vi "DriveVelocityHeadingFollower.vi"(0 "RobotMotors":T20={"DriveLeftPrimary"={"DeviceStatus"={"status"=FALSE, "code"=0, "source"=""}, "Type"=enum."PWM", "PWM"={"PWM Channel"=enum."PWM 1", "DeadBand"={"Name"="", "maxPositivePwm"=0, "minPositivePwm"=0, "centerPwm"=0, "maxNegativePwm"=0, "minNegativePwm"=0, "angularRange"=0}}, "CAN"={"Device Number"=0, "SetOutput VI Ref"=variant(enum8{"Percent VBus", "Current", "Speed", "Position", "Voltage"} enum."Percent VBus"), "GetOutput VI Ref"=variant(refnum<k1> refnum), "Enable VI Ref"=variant(dbl 12.0), "Disable VI Ref"=variant(enum8{"Percent VBus", "Speed", "Position", "Slave", "Unchanged / Invalid", "Voltage Compensation", "Current", "Motion Profile"} enum."Percent VBus"), "Data"=variant}, "Invert"=FALSE, "DIO PWM"={"PWM \"Enable\" Channel"=enum."Invalid", "DIOChannel"=enum."Invalid", "PWM Rate"=0.0}}, "DriveLeftSecondary1"={"DeviceStatus"={"status"=FALSE, "code"=0, "source"=""}, "Type"=enum."PWM", "PWM"={"PWM Channel"=enum."PWM 1", "DeadBand"={"Name"="", "maxPositivePwm"=0, "minPositivePwm"=0, "centerPwm"=0, "maxNegativePwm"=0, "minNegativePwm"=0, "angularRange"=0}}, "CAN"={"Device Number"=0, "SetOutput VI Ref"=variant(enum8{"Percent VBus", "Current", "Speed", "Position", "Voltage"} enum."Percent VBus"), "GetOutput VI Ref"=variant(refnum<k1> refnum), "Enable VI Ref"=variant(dbl 12.0), "Disable VI Ref"=variant(enum8{"Percent VBus", "Speed", "Position", "Slave", "Unchanged / Invalid", "Voltage Compensation", "Current", "Motion Profile"} enum."Percent VBus"), "Data"=variant}, "Invert"=FALSE, "DIO PWM"={"PWM \"Enable\" Channel"=enum."Invalid", "DIOChannel"=enum."Invalid", "PWM Rate"=0.0}}, "DriveRightPrimary"={"DeviceStatus"={"status"=FALSE, "code"=0, "source"=""}, "Type"=enum."PWM", "PWM"={"PWM Channel"=enum."PWM 1", "DeadBand"={"Name"="", "maxPositivePwm"=0, "minPositivePwm"=0, "centerPwm"=0, "maxNegativePwm"=0, "minNegativePwm"=0, "angularRange"=0}}, "CAN"={"Device Number"=0, "SetOutput VI Ref"=variant(enum8{"Percent VBus", "Current", "Speed", "Position", "Voltage"} enum."Percent VBus"), "GetOutput VI Ref"=variant(refnum<k1> refnum), "Enable VI Ref"=variant(dbl 12.0), "Disable VI Ref"=variant(enum8{"Percent VBus", "Speed", "Position", "Slave", "Unchanged / Invalid", "Voltage Compensation", "Current", "Motion Profile"} enum."Percent VBus"), "Data"=variant}, "Invert"=FALSE, "DIO PWM"={"PWM \"Enable\" Channel"=enum."Invalid", "DIOChannel"=enum."Invalid", "PWM Rate"=0.0}}, "DriveRightSecondary1"={"DeviceStatus"={"status"=FALSE, "code"=0, "source"=""}, "Type"=enum."PWM", "PWM"={"PWM Channel"=enum."PWM 1", "DeadBand"={"Name"="", "maxPositivePwm"=0, "minPositivePwm"=0, "centerPwm"=0, "maxNegativePwm"=0, "minNegativePwm"=0, "angularRange"=0}}, "CAN"={"Device Number"=0, "SetOutput VI Ref"=variant(enum8{"Percent VBus", "Current", "Speed", "Position", "Voltage"} enum."Percent VBus"), "GetOutput VI Ref"=variant(refnum<k1> refnum), "Enable VI Ref"=variant(dbl 12.0), "Disable VI Ref"=variant(enum8{"Percent VBus", "Speed", "Position", "Slave", "Unchanged / Invalid", "Voltage Compensation", "Current", "Motion Profile"} enum."Percent VBus"), "Data"=variant}, "Invert"=FALSE, "DIO PWM"={"PWM \"Enable\" Channel"=enum."Invalid", "DIOChannel"=enum."Invalid", "PWM Rate"=0.0}}, " RightIntake"={"DeviceStatus"={"status"=FALSE, "code"=0, "source"=""}, "Type"=enum."PWM", "PWM"={"PWM Channel"=enum."PWM 1", "DeadBand"={"Name"="", "maxPositivePwm"=0, "minPositivePwm"=0, "centerPwm"=0, "maxNegativePwm"=0, "minNegativePwm"=0, "angularRange"=0}}, "CAN"={"Device Number"=0, "SetOutput VI Ref"=variant(enum8{"Percent VBus", "Current", "Speed", "Position", "Voltage"} enum."Percent VBus"), "GetOutput VI Ref"=variant(refnum<k1> refnum), "Enable VI Ref"=variant(dbl 12.0), "Disable VI Ref"=variant(enum8{"Percent VBus", "Speed", "Position", "Slave", "Unchanged / Invalid", "Voltage Compensation", "Current", "Motion Profile"} enum."Percent VBus"), "Data"=variant}, "Invert"=FALSE, "DIO PWM"={"PWM \"Enable\" Channel"=enum."Invalid", "DIOChannel"=enum."Invalid", "PWM Rate"=0.0}}, "LeftIntake"={"DeviceStatus"={"status"=FALSE, "code"=0, "source"=""}, "Type"=enum."PWM", "PWM"={"PWM Channel"=enum."PWM 1", "DeadBand"={"Name"="", "maxPositivePwm"=0, "minPositivePwm"=0, "centerPwm"=0, "maxNegativePwm"=0, "minNegativePwm"=0, "angularRange"=0}}, "CAN"={"Device Number"=0, "SetOutput VI Ref"=variant(enum8{"Percent VBus", "Current", "Speed", "Position", "Voltage"} enum."Percent VBus"), "GetOutput VI Ref"=variant(refnum<k1> refnum), "Enable VI Ref"=variant(dbl 12.0), "Disable VI Ref"=variant(enum8{"Percent VBus", "Speed", "Position", "Slave", "Unchanged / Invalid", "Voltage Compensation", "Current", "Motion Profile"} enum."Percent VBus"), "Data"=variant}, "Invert"=FALSE, "DIO PWM"={"PWM \"Enable\" Channel"=enum."Invalid", "DIOChannel"=enum."Invalid", "PWM Rate"=0.0}}, "ArmPivot"={"DeviceStatus"={"status"=FALSE, "code"=0, "source"=""}, "Type"=enum."PWM", "PWM"={"PWM Channel"=enum."PWM 1", "DeadBand"={"Name"="", "maxPositivePwm"=0, "minPositivePwm"=0, "centerPwm"=0, "maxNegativePwm"=0, "minNegativePwm"=0, "angularRange"=0}}, "CAN"={"Device Number"=0, "SetOutput VI Ref"=variant(enum8{"Percent VBus", "Current", "Speed", "Position", "Voltage"} enum."Percent VBus"), "GetOutput VI Ref"=variant(refnum<k1> refnum), "Enable VI Ref"=variant(dbl 12.0), "Disable VI Ref"=variant(enum8{"Percent VBus", "Speed", "Position", "Slave", "Unchanged / Invalid", "Voltage Compensation", "Current", "Motion Profile"} enum."Percent VBus"), "Data"=variant}, "Invert"=FALSE, "DIO PWM"={"PWM \"Enable\" Channel"=enum."Invalid", "DIOChannel"=enum."Invalid", "PWM Rate"=0.0}}, "ArmPivot 2 "={"DeviceStatus"={"status"=FALSE, "code"=0, "source"=""}, "Type"=enum."PWM", "PWM"={"PWM Channel"=enum."PWM 1", "DeadBand"={"Name"="", "maxPositivePwm"=0, "minPositivePwm"=0, "centerPwm"=0, "maxNegativePwm"=0, "minNegativePwm"=0, "angularRange"=0}}, "CAN"={"Device Number"=0, "SetOutput VI Ref"=variant(enum8{"Percent VBus", "Current", "Speed", "Position", "Voltage"} enum."Percent VBus"), "GetOutput VI Ref"=variant(refnum<k1> refnum), "Enable VI Ref"=variant(dbl 12.0), "Disable VI Ref"=variant(enum8{"Percent VBus", "Speed", "Position", "Slave", "Unchanged / Invalid", "Voltage Compensation", "Current", "Motion Profile"} enum."Percent VBus"), "Data"=variant}, "Invert"=FALSE, "DIO PWM"={"PWM \"Enable\" Channel"=enum."Invalid", "DIOChannel"=enum."Invalid", "PWM Rate"=0.0}}, "ArmExtend "={"DeviceStatus"={"status"=FALSE, "code"=0, "source"=""}, "Type"=enum."PWM", "PWM"={"PWM Channel"=enum."PWM 1", "DeadBand"={"Name"="", "maxPositivePwm"=0, "minPositivePwm"=0, "centerPwm"=0, "maxNegativePwm"=0, "minNegativePwm"=0, "angularRange"=0}}, "CAN"={"Device Number"=0, "SetOutput VI Ref"=variant(enum8{"Percent VBus", "Current", "Speed", "Position", "Voltage"} enum."Percent VBus"), "GetOutput VI Ref"=variant(refnum<k1> refnum), "Enable VI Ref"=variant(dbl 12.0), "Disable VI Ref"=variant(enum8{"Percent VBus", "Speed", "Position", "Slave", "Unchanged / Invalid", "Voltage Compensation", "Current", "Motion Profile"} enum."Percent VBus"), "Data"=variant}, "Invert"=FALSE, "DIO PWM"={"PWM \"Enable\" Channel"=enum."Invalid", "DIOChannel"=enum."Invalid", "PWM Rate"=0.0}}, "Climber"={"DeviceStatus"={"status"=FALSE, "code"=0, "source"=""}, "Type"=enum."PWM", "PWM"={"PWM Channel"=enum."PWM 1", "DeadBand"={"Name"="", "maxPositivePwm"=0, "minPositivePwm"=0, "centerPwm"=0, "maxNegativePwm"=0, "minNegativePwm"=0, "angularRange"=0}}, "CAN"={"Device Number"=0, "SetOutput VI Ref"=variant(enum8{"Percent VBus", "Current", "Speed", "Position", "Voltage"} enum."Percent VBus"), "GetOutput VI Ref"=variant(refnum<k1> refnum), "Enable VI Ref"=variant(dbl 12.0), "Disable VI Ref"=variant(enum8{"Percent VBus", "Speed", "Position", "Slave", "Unchanged / Invalid", "Voltage Compensation", "Current", "Motion Profile"} enum."Percent VBus"), "Data"=variant}, "Invert"=FALSE, "DIO PWM"={"PWM \"Enable\" Channel"=enum."Invalid", "DIOChannel"=enum."Invalid", "PWM Rate"=0.0}}, "SelfieStick"={"DeviceStatus"={"status"=FALSE, "code"=0, "source"=""}, "Type"=enum."PWM", "PWM"={"PWM Channel"=enum."PWM 1", "DeadBand"={"Name"="", "maxPositivePwm"=0, "minPositivePwm"=0, "centerPwm"=0, "maxNegativePwm"=0, "minNegativePwm"=0, "angularRange"=0}}, "CAN"={"Device Number"=0, "SetOutput VI Ref"=variant(enum8{"Percent VBus", "Current", "Speed", "Position", "Voltage"} enum."Percent VBus"), "GetOutput VI Ref"=variant(refnum<k1> refnum), "Enable VI Ref"=variant(dbl 12.0), "Disable VI Ref"=variant(enum8{"Percent VBus", "Speed", "Position", "Slave", "Unchanged / Invalid", "Voltage Compensation", "Current", "Motion Profile"} enum."Percent VBus"), "Data"=variant}, "Invert"=FALSE, "DIO PWM"={"PWM \"Enable\" Channel"=enum."Invalid", "DIOChannel"=enum."Invalid", "PWM Rate"=0.0}}}, 1 "RobotConfig":T3={"Motors"={"DriveLeftPrimary"={"CAN Address"=1, "Invert"=FALSE, "InvertSensor"=FALSE, "Unit Conversion Factor"=0.0, "Brake Mode"=enum."Override to Brake", "Reverse Limt Switch Mode"=enum."Normally Closed", "Forward Limt Swith Mode"=enum."Normally Closed", "PWM Channel"=enum."Invalid", "Motor Controller Type"=enum."Talon SRX"}, "DriveLeftSecondary1"={"CAN Address"=2, "Invert"=FALSE, "InvertSensor"=FALSE, "Unit Conversion Factor"=0.0, "Brake Mode"=enum."Override to Brake", "Reverse Limt Switch Mode"=enum."Normally Closed", "Forward Limt Swith Mode"=enum."Normally Closed", "PWM Channel"=enum."Invalid", "Motor Controller Type"=enum."Talon SRX"}, "DriveRightPrimary"={"CAN Address"=3, "Invert"=FALSE, "InvertSensor"=FALSE, "Unit Conversion Factor"=0.0, "Brake Mode"=enum."Override to Brake", "Reverse Limt Switch Mode"=enum."Normally Closed", "Forward Limt Swith Mode"=enum."Normally Closed", "PWM Channel"=enum."Invalid", "Motor Controller Type"=enum."Talon SRX"}, "DriveRightSecondary1"={"CAN Address"=4, "Invert"=FALSE, "InvertSensor"=FALSE, "Unit Conversion Factor"=0.0, "Brake Mode"=enum."Override to Brake", "Reverse Limt Switch Mode"=enum."Normally Closed", "Forward Limt Swith Mode"=enum."Normally Closed", "PWM Channel"=enum."Invalid", "Motor Controller Type"=enum."Talon SRX"}, "RightIntake"={"CAN Address"=8, "Invert"=FALSE, "InvertSensor"=FALSE, "Unit Conversion Factor"=0.0, "Brake Mode"=enum."Override to Brake", "Reverse Limt Switch Mode"=enum."Normally Closed", "Forward Limt Swith Mode"=enum."Normally Closed", "PWM Channel"=enum."Invalid", "Motor Controller Type"=enum."Talon SRX"}, "LeftIntake"={"CAN Address"=7, "Invert"=FALSE, "InvertSensor"=FALSE, "Unit Conversion Factor"=0.0, "Brake Mode"=enum."Override to Brake", "Reverse Limt Switch Mode"=enum."Normally Closed", "Forward Limt Swith Mode"=enum."Normally Closed", "PWM Channel"=enum."Invalid", "Motor Controller Type"=enum."Talon SRX"}, "ArmPivot"={"CAN Address"=5, "Invert"=FALSE, "InvertSensor"=FALSE, "Unit Conversion Factor"=0.0, "Brake Mode"=enum."Override to Brake", "Reverse Limt Switch Mode"=enum."Normally Closed", "Forward Limt Swith Mode"=enum."Normally Closed", "PWM Channel"=enum."Invalid", "Motor Controller Type"=enum."Talon SRX"}, "ArmExtend"={"CAN Address"=6, "Invert"=FALSE, "InvertSensor"=FALSE, "Unit Conversion Factor"=0.0, "Brake Mode"=enum."Override to Brake", "Reverse Limt Switch Mode"=enum."Normally Closed", "Forward Limt Swith Mode"=enum."Normally Closed", "PWM Channel"=enum."Invalid", "Motor Controller Type"=enum."Talon SRX"}, "ArmPivot2"={"CAN Address"=9, "Invert"=FALSE, "InvertSensor"=FALSE, "Unit Conversion Factor"=0.0, "Brake Mode"=enum."Override to Brake", "Reverse Limt Switch Mode"=enum."Normally Closed", "Forward Limt Swith Mode"=enum."Normally Closed", "PWM Channel"=enum."Invalid", "Motor Controller Type"=enum."Talon SRX"}, "Climber"={"CAN Address"=10, "Invert"=FALSE, "InvertSensor"=FALSE, "Unit Conversion Factor"=0.0, "Brake Mode"=enum."Override to Brake", "Reverse Limt Switch Mode"=enum."Disabled", "Forward Limt Swith Mode"=enum."Disabled", "PWM Channel"=enum."Invalid", "Motor Controller Type"=enum."Talon SRX"}, "Selfie Stick"={"CAN Address"=11, "Invert"=FALSE, "InvertSensor"=FALSE, "Unit Conversion Factor"=0.0, "Brake Mode"=enum."Override to Brake", "Reverse Limt Switch Mode"=enum."Disabled", "Forward Limt Swith Mode"=enum."Disabled", "PWM Channel"=enum."Invalid", "Motor Controller Type"=enum."Talon SRX"}}, "Sensors"={"IMU"={"Yaw Axis"=enum."Z", "SPI Bus"=enum."SPI MXP", "AHRS Algorithm"=enum."Complementary", "Calibration Time (s)"=3.0, "Calibrate On Open"=TRUE}, "LimitSwitch1"={"DIOChannel"=enum."DIO 0", "Active Low"=FALSE}, "LimitSwitch2"={"DIOChannel"=enum."DIO 1", "Active Low"=FALSE}, "BeamBreak"={"DIOChannel"=enum."DIO 2", "Active Low"=FALSE}, "JeVois"={"Baud Rate"=9600, "Parity"=0, "Data Bits"=8, "Stop Bits"=10, "Termination Char (0xA = '\\n' = LF)"=10, "Enable Termination Char? (T)"=TRUE, "Flow Control"=0, "Timeout Value (ms)"=5000, "Serial Port"=enum."Onboard RS-232"}}, "PID"={"ArmExtend"={"P"=0.0, "I"=0.0, "D"=0.0, "F"=0.0, "IZone"=0.0}, "ArmRotate"={"P"=0.0, "I"=0.0, "D"=0.0, "F"=0.0, "IZone"=0.0}, "Drive"={"P"=0.0, "I"=0.0, "D"=0.0, "F"=0.0, "IZone"=0.0}, "DriveGyro Kp ((in/sec)/deg)"=0.0, "CameraPole"={"P"=0.0, "I"=0.0, "D"=0.0, "F"=0.0, "IZone"=0.0}}, "Solenoids"={"ArmClaw"={"Forward Channel"=enum."Solenoid 0", "Invert"=FALSE, "Reverse Channel"=enum."Solenoid 0"}, "IntakeExtend"={"Forward Channel"=enum."Solenoid 1", "Invert"=FALSE, "Reverse Channel"=enum."Solenoid 0"}, "IntakeOpen"={"Forward Channel"=enum."Solenoid 2", "Invert"=FALSE, "Reverse Channel"=enum."Solenoid 0"}, " Shifter"={"Forward Channel"=enum."Solenoid 3", "Invert"=FALSE, "Reverse Channel"=enum."Solenoid 0"}}, "RobotDimensions "={"Length"=0.0, "Height"=0.0, "HeightOfBumpers"=0.0, "DistanceFromFrameEdgeToPyramid "=0.0, "HeightOfFrameToIntake"=0.0, "EdgeOfFrameToOrigin"=0.0}, "ArmHomePosition"={"Angle (rad)"=0.0, "Radius (in)"=0.0}, "SelfieStickParams"={"Home Height (in)"=0.0, "CruiseVelocity"=0, "MaxAccel"=0, "Low Height (in)"=0.0, "High Height (in)"=0.0, "Mid Height (in)"=0.0}, "Enable Compressor"=TRUE} {"Sensors"."JeVois"."Flow Control" items=["None", "XON/XOFF", "RTS/CTS", "XON/XOFF & RTS/CTS", "DTR/DSR", "XON/XOFF & DTR/DSR"]; "Sensors"."JeVois"."Termination Char (0xA = '\\n' = LF)" format="%.0x"; "Sensors"."JeVois"."Stop Bits" items=["1.0"=10, "1.5"=15, "2.0"=20]; "Sensors"."JeVois"."Parity" items=["None", "Odd", "Even", "Mark", "Space"]}, 2 "IMU DevRef":T1={"DevStatus"={"status"=FALSE, "code"=0, "source"=""}, "Handle"=0, "SPI Bus"=enum."SPI On-Board, CS0", "Device Found"=FALSE, "Device Ready"=FALSE, "Yaw Axis"=enum."Z", "AHRS Algorithm"=enum."Complementary", "Serial"=0, "Lot ID 2"=0, "Lot ID 1"=0, "Bytes Per Sample"=0, "Calibrate On Open?"=FALSE}, 3 "DriveCompleteNotifier":refnum<notifier>, 4 "DriveGyro Kp ((in/sec)/deg)":dbl) -> ()   [LabVIEW 2017]
uses:
  TypeDefs/RobotComponents/RobotMotors.ctl
  <vilib>/Rock Robotics/WPI/MotorControl/WPI_MotorControlDeviceRef.ctl
  <vilib>/Rock Robotics/WPI/MotorControl/WPI_MotorControlType.ctl
  <vilib>/Rock Robotics/SystemInterfaces/DIO/FPGA_DIOPWMChannel.ctl
  <vilib>/Rock Robotics/WPI/PWM/WPI_PWMDeadband.ctl
  <vilib>/Rock Robotics/SystemInterfaces/DIO/FPGA_DIOChannel.ctl
  TypeDefs/ConfigComponents/Config_Robot.ctl
  ArgosLib/Config/ConfigComponents/TypeDefs/Config_Motor.ctl
  <vilib>/Rock Robotics/WPI/ThirdParty/Phoenix-LabVIEW/Motor Controller/Controls/CTRE_Phoenix_MotorControl_NeutralMode.ctl
  <vilib>/Rock Robotics/WPI/ThirdParty/Phoenix-LabVIEW/Motor Controller/Controls/CTRE_Phoenix_MotorControl_LimitSwitchNormal.ctl
  ArgosLib/Config/ConfigComponents/TypeDefs/Config_MotorCtrlType.ctl
  ArgosLib/Config/ConfigComponents/TypeDefs/Config_IMU.ctl
  <vilib>/Rock Robotics/SystemInterfaces/spilib/spi_bus.ctl
  ArgosLib/Config/ConfigComponents/TypeDefs/Config_DigitalIO.ctl
  ArgosLib/Config/ConfigComponents/TypeDefs/Config_SerialPort.ctl
  <vilib>/Rock Robotics/WPI/SerialPort/WPI_SerialPort.ctl
  ArgosLib/Config/ConfigComponents/TypeDefs/Config_PIDParams.ctl
  ArgosLib/Config/ConfigComponents/TypeDefs/Config_DoubleSolenoid.ctl
  <vilib>/Rock Robotics/WPI/Solenoid/WPI_SolenoidChannel.ctl
  TypeDefs/ConfigComponents/Config_Dimensions.ctl
  TypeDefs/ConfigComponents/Config_ArmHome.ctl
  TypeDefs/ConfigComponents/Config_SelfieStick.ctl
  Sensors/IMU/ADI_IMU_ADIS16448_IMUDevRef.ctl
  ArgosLib/Signal Processing/TypeDefs/EdgeDetector_Type.ctl
  <vilib>/Rock Robotics/WPI/ThirdParty/Phoenix-LabVIEW/Motor Controller/Controls/CTRE_Phoenix_MotorControl_ControlMode.ctl
  Global_Var-RefNum/MotionProfileControlData.vi
  Sensors/IMU/ADIS16448_IMU.lvlib
  ArgosLib/ArgosLib.lvlib
panel:
  in  "MinCompletionPercent":dbl=0.5
  in  "Stopped Velocity Threshold (in/sec)":dbl=1.0
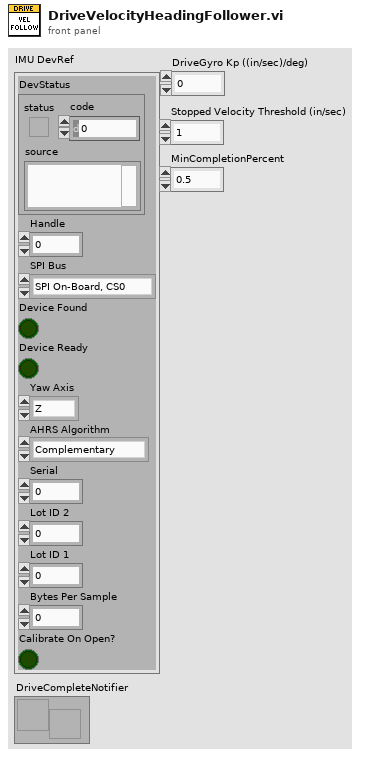
[diagram p1: front panel]
types:
  T1 = typedef "ADIS16448_IMU.lvlib/ADI_IMU_ADIS16448_IMUDevRef.ctl" = cluster{"DevStatus":errorcluster, "Handle":i32, "SPI Bus":T2, "Device Found":bool, "Device Ready":bool, "Yaw Axis":enum16{"X", "Y", "Z"}, "AHRS Algorithm":enum16{"Complementary", "Madgwick"}, "Serial":u16, "Lot ID 2":u16, "Lot ID 1":u16, "Bytes Per Sample":u16, "Calibrate On Open?":bool}
  T2 = typedef "spi_bus.ctl" = enum16{"SPI On-Board, CS0", "SPI On-Board, CS1", "SPI On-Board, CS2", "SPI On-Board, CS3", "SPI MXP", "Invalid"}
  T3 = typedef "Config_Robot.ctl" = cluster{"Motors":cluster{"DriveLeftPrimary":T4, "DriveLeftSecondary1":T4, "DriveRightPrimary":T4, "DriveRightSecondary1":T4, "RightIntake":T4, "LeftIntake":T4, "ArmPivot":T4, "ArmExtend":T4, "ArmPivot2":T4, "Climber":T4, "Selfie Stick":T4}, "Sensors":cluster{"IMU":T9, "LimitSwitch1":T10, "LimitSwitch2":T10, "BeamBreak":T10, "JeVois":T12}, "PID":cluster{"ArmExtend":T14, "ArmRotate":T14, "Drive":T14, "DriveGyro Kp ((in/sec)/deg)":dbl, "CameraPole":T14}, "Solenoids":cluster{"ArmClaw":T15, "IntakeExtend":T15, "IntakeOpen":T15, " Shifter":T15}, "RobotDimensions ":T17, "ArmHomePosition":T18, "SelfieStickParams":T19, "Enable Compressor":bool}
  T4 = typedef "Config_Motor.ctl" = cluster{"CAN Address":u8, "Invert":bool, "InvertSensor":bool, "Unit Conversion Factor":dbl, "Brake Mode":T5, "Reverse Limt Switch Mode":T6, "Forward Limt Swith Mode":T6, "PWM Channel":T7, "Motor Controller Type":T8}
  T5 = typedef "CTRE_Phoenix_MotorControl_NeutralMode.ctl" = enum8{"EEPROMSetting", "Override to Coast", "Override to Brake"}
  T6 = typedef "CTRE_Phoenix_MotorControl_LimitSwitchNormal.ctl" = enum16{"Normally Open", "Normally Closed", "Disabled"}
  T7 = typedef "FPGA_DIOPWMChannel.ctl" = enum8{"PWM 0", "PWM 1", "PWM 2", "PWM 3", "PWM 4", "PWM 5", "PWM 6", "PWM 7", "PWM 8", "PWM 9", "PWM MXP 0", "PWM MXP 1", "PWM MXP 2", "PWM MXP 3", "PWM MXP 4", "PWM MXP 5", "PWM MXP 6", "PWM MXP 7", "PWM MXP 8", "PWM MXP 9", "Invalid"}
  T8 = typedef "Config_MotorCtrlType.ctl" = enum16{"Disabled", "Talon SRX", "Talon SR"}
  T9 = typedef "Config_IMU.ctl" = cluster{"Yaw Axis":enum16{"X", "Y", "Z"}, "SPI Bus":T2, "AHRS Algorithm":enum16{"Complementary", "Madgwick"}, "Calibration Time (s)":dbl, "Calibrate On Open":bool}
  T10 = typedef "Config_DigitalIO.ctl" = cluster{"DIOChannel":T11, "Active Low":bool}
  T11 = typedef "FPGA_DIOChannel.ctl" = enum8{"DIO 0", "DIO 1", "DIO 2", "DIO 3", "DIO 4", "DIO 5", "DIO 6", "DIO 7", "DIO 8", "DIO 9", "DIO MXP 0", "DIO MXP 1", "DIO MXP 2", "DIO MXP 3", "DIO MXP 4", "DIO MXP 5", "DIO MXP 6", "DIO MXP 7", "DIO MXP 8", "DIO MXP 9", "DIO MXP 10", "DIO MXP 11", "DIO MXP 12", "DIO MXP 13", "DIO MXP 14", "DIO MXP 15", "SPI Port CS1", "SPI Port CS2", "SPI Port CS3", "SPI Port MISO", "SPI Port MOSI", "Invalid"}
  T12 = typedef "Config_SerialPort.ctl" = cluster{"Baud Rate":u32, "Parity":u16, "Data Bits":u16, "Stop Bits":u16, "Termination Char (0xA = '\\n' = LF)":u8, "Enable Termination Char? (T)":bool, "Flow Control":u16, "Timeout Value (ms)":u32, "Serial Port":T13}
  T13 = typedef "WPI_SerialPort.ctl" = enum16{"Onboard RS-232", "MXP TTL", "USB 1", "USB 2"}
  T14 = typedef "Config_PIDParams.ctl" = cluster{"P":dbl, "I":dbl, "D":dbl, "F":dbl, "IZone":dbl}
  T15 = typedef "Config_DoubleSolenoid.ctl" = cluster{"Forward Channel":T16, "Invert":bool, "Reverse Channel":T16}
  T16 = typedef "WPI_SolenoidChannel.ctl" = enum8{"Solenoid 0", "Solenoid 1", "Solenoid 2", "Solenoid 3", "Solenoid 4", "Solenoid 5", "Solenoid 6", "Solenoid 7", "Invalid"}
  T17 = typedef "Config_Dimensions.ctl" = cluster{"Length":dbl, "Height":dbl, "HeightOfBumpers":dbl, "DistanceFromFrameEdgeToPyramid ":dbl, "HeightOfFrameToIntake":dbl, "EdgeOfFrameToOrigin":dbl}
  T18 = typedef "Config_ArmHome.ctl" = cluster{"Angle (rad)":dbl, "Radius (in)":dbl}
  T19 = typedef "Config_SelfieStick.ctl" = cluster{"Home Height (in)":dbl, "CruiseVelocity":i32, "MaxAccel":i32, "Low Height (in)":dbl, "High Height (in)":dbl, "Mid Height (in)":dbl}
  T20 = typedef "RobotMotors.ctl" = cluster{"DriveLeftPrimary":T21, "DriveLeftSecondary1":T21, "DriveRightPrimary":T21, "DriveRightSecondary1":T21, " RightIntake":T21, "LeftIntake":T21, "ArmPivot":T21, "ArmPivot 2 ":T21, "ArmExtend ":T21, "Climber":T21, "SelfieStick":T21}
  T21 = typedef "WPI_MotorControlDeviceRef.ctl" = cluster{"DeviceStatus":errorcluster, "Type":T22, "PWM":cluster{"PWM Channel":T7, "DeadBand":T23}, "CAN":cluster{"Device Number":u8, "SetOutput VI Ref":variant, "GetOutput VI Ref":variant, "Enable VI Ref":variant, "Disable VI Ref":variant, "Data":variant}, "Invert":bool, "DIO PWM":cluster{"PWM \"Enable\" Channel":T7, "DIOChannel":T11, "PWM Rate":dbl}}
  T22 = typedef "WPI_MotorControlType.ctl" = enum16{"PWM", "CAN", "DIO PWM"}
  T23 = typedef "WPI_PWMDeadband.ctl" = cluster{"Name":string, "maxPositivePwm":i32, "minPositivePwm":i32, "centerPwm":i32, "maxNegativePwm":i32, "minNegativePwm":i32, "angularRange":u16}
  T24 = typedef "ArgosLib.lvlib/EdgeDetector_Type.ctl" = enum16{"RisingEdge", "FallingEdge", "Both"}
  T25 = typedef "DriveMotionProfileControl.ctl" = cluster{"ControlMutex":T26, "Trajectory Points":T27[], "CurrentIndex":u32}
  T26 = typedef "Semaphore RefNum" = refnum<k1>
  T27 = typedef "Pathfinder.lvlib/Segment.ctl" = cluster{"dt":dbl, "x":dbl, "y":dbl, "position":dbl, "velocity":dbl, "acceleration":dbl, "jerk":dbl, "heading":dbl}
  T28 = cluster{"X Angle":dbl, "Y Angle":dbl, "Z Angle":dbl}
  T29 = typedef "CTRE_Phoenix_MotorControl_ControlMode.ctl" = u16
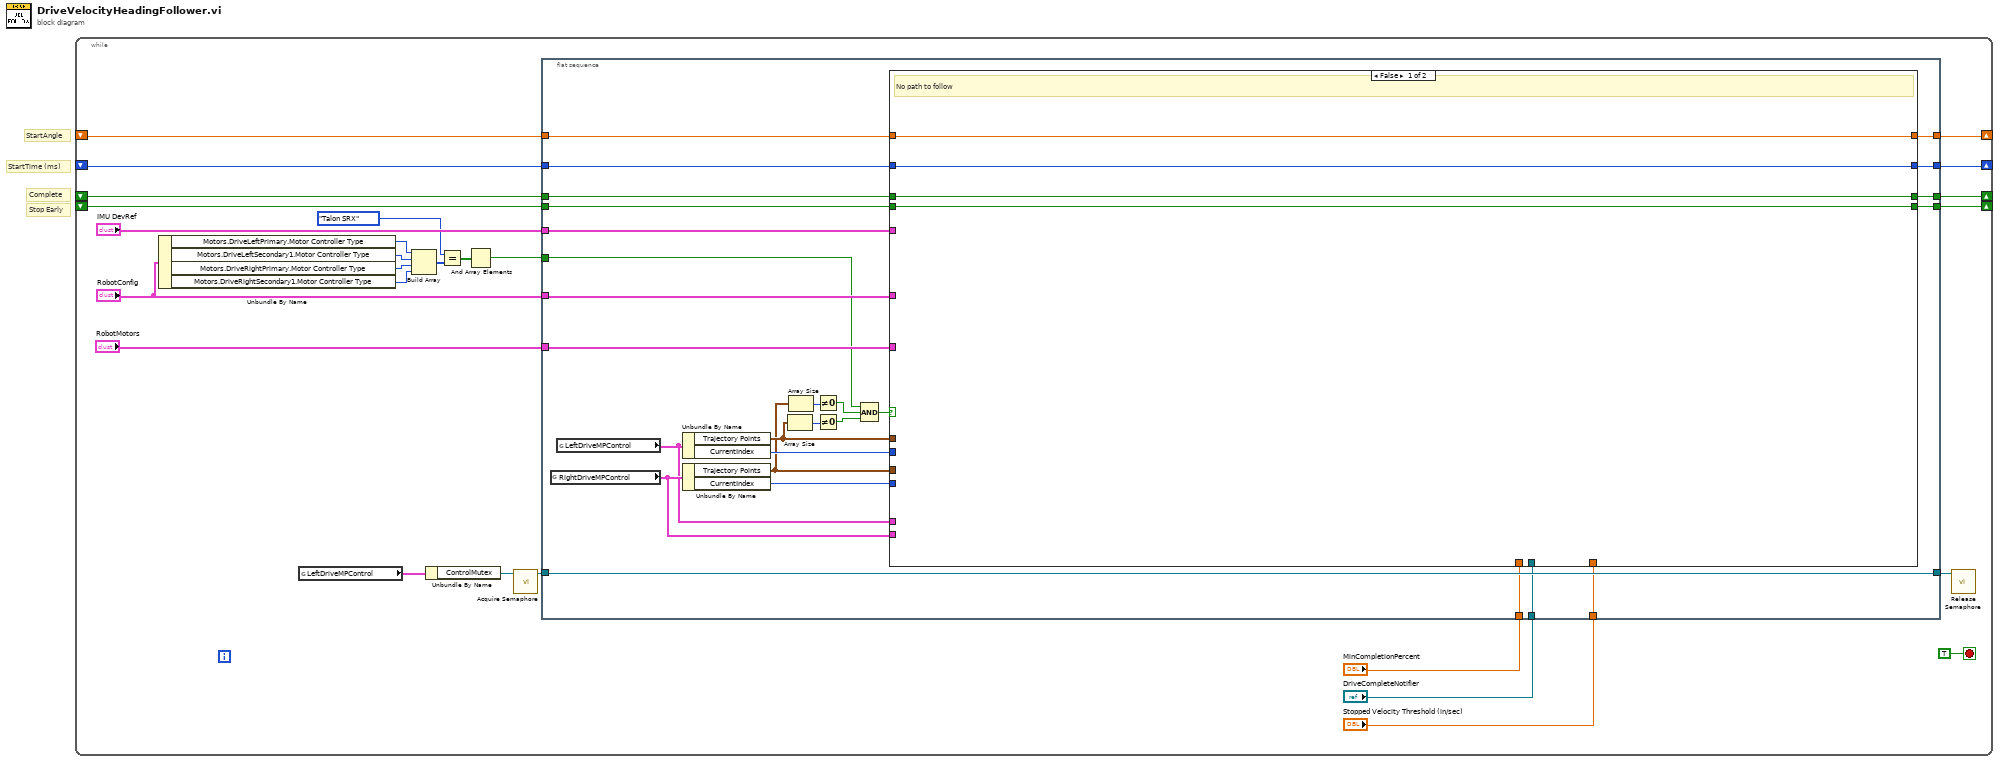
[diagram p0: block diagram]
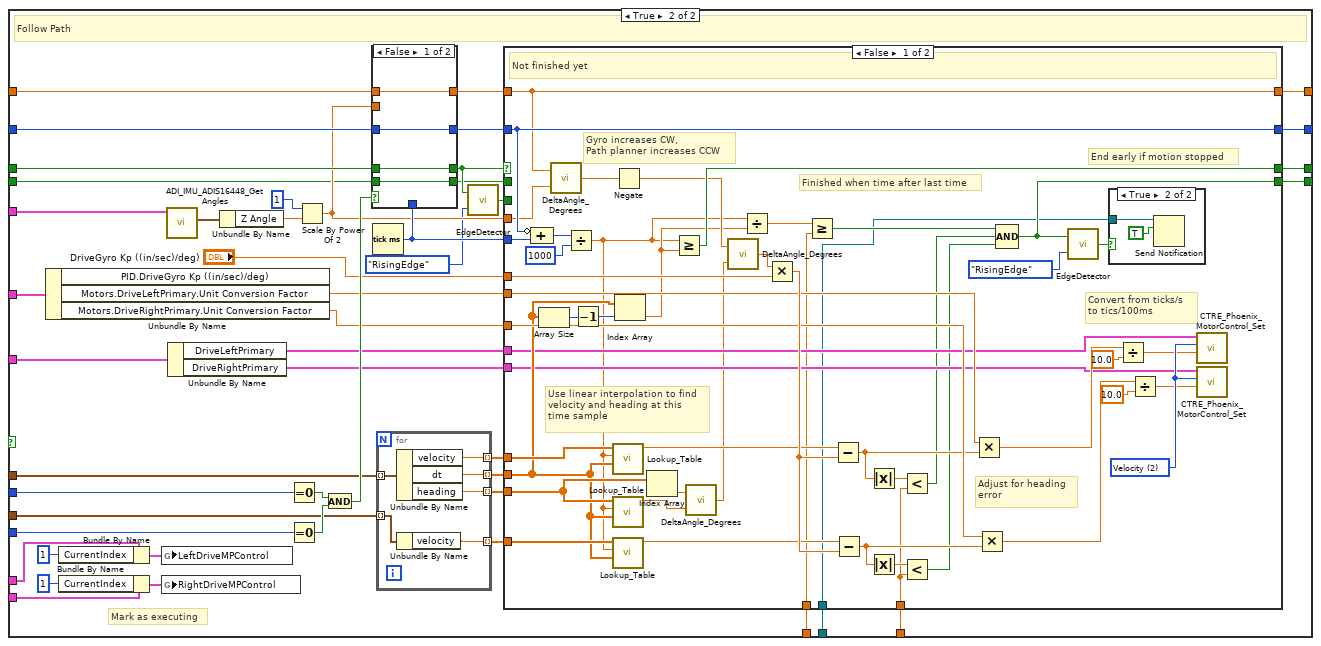
[diagram p2: hidden frame]
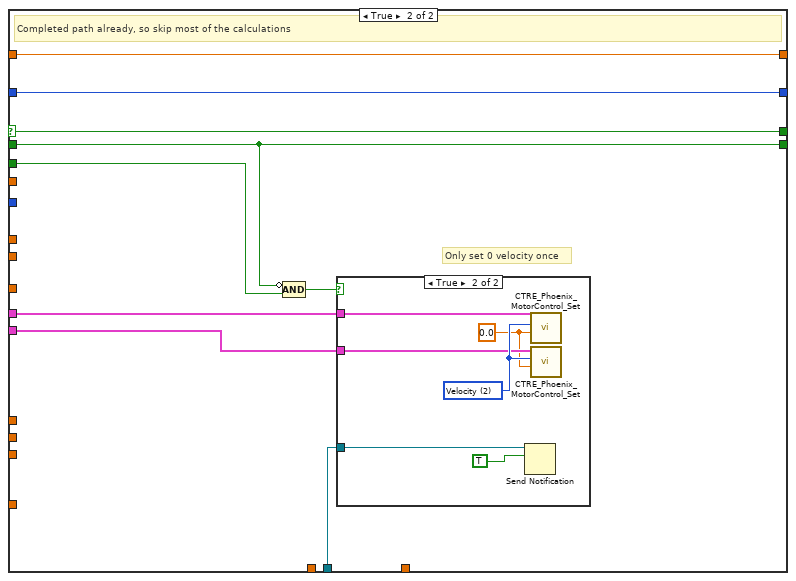
[diagram p4: hidden frame]
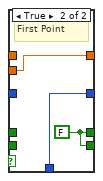
[diagram p6: hidden frame]
diagram:
  # "Stop Early"
  # "Complete"
  # "StartAngle"
  # "StartTime (ms)"
  n1 = while {
    shift-right: [w19] -> _
    shift-left: _ -> [w20]
    shift-right: [w18] -> _
    shift-left: _ -> [w17]
    shift-right: [w15] -> _
    shift-left: _ -> [w16]
    shift-right: [w14] -> _
    shift-left: _ -> [w13]
    stop <- TRUE stop-if-true
    n2 = Unbundle By Name("RobotConfig") -> ("Motors.DriveLeftPrimary.Motor Controller Type"=w8:T8, "Motors.DriveLeftSecondary1.Motor Controller Type"=w7:T8, "Motors.DriveRightPrimary.Motor Controller Type"=w6:T8, "Motors.DriveRightSecondary1.Motor Controller Type"=w5:T8)
    n3 = global read "MotionProfileControlData.vi" "LeftDriveMPControl"() -> (w24:T25)
    n4 = Build Array(w8, w7, w6, w5) -> (w4:T8[])
    n5 = Unbundle By Name(w24) -> ("ControlMutex"=w27:T26)
    n6 = Equal?(x=Config_MotorCtrlType."Talon SRX" ("Motors.DriveLeftPrimary.Motor Controller Type"), y=w4) -> (x = y?=w2:bool[])
    n7 = And Array Elements(Boolean array=w2) -> (logical AND=w1:bool)
    n8 = call <vilib>:"Acquire Semaphore.vi"("semaphore"=w27) -> ("semaphore out"=w26:T26)  [unwired: 4 in, 2 out]
    n9 = flat-sequence {
      tunnel: w26 -> [w54]
      tunnel: [w54] -> w25
      tunnel: "IMU DevRef" -> [w53]
      tunnel: "RobotMotors" -> [w52]
      tunnel: "RobotConfig" -> [w51]
      tunnel: w20 -> [w48]
      tunnel: [w45] -> w19
      tunnel: [w46] -> w18
      tunnel: w17 -> [w47]
      tunnel: w16 -> [w37]
      tunnel: [w36] -> w15
      tunnel: [w35] -> w14
      tunnel: w13 -> [w34]
      tunnel: "DriveCompleteNotifier" -> [w33]
      tunnel: "Stopped Velocity Threshold (in/sec)" -> [w32]
      tunnel: "MinCompletionPercent" -> [w31]
      tunnel: w1 -> [w28]
      frame #0 {
        n10 = global read "MotionProfileControlData.vi" "RightDriveMPControl"() -> (w30:T25)
        n11 = global read "MotionProfileControlData.vi" "LeftDriveMPControl"() -> (w29:T25)
        n12 = Unbundle By Name(w29) -> ("Trajectory Points"=w44:T27[], "CurrentIndex"=w50:u32)
        n13 = Unbundle By Name(w30) -> ("Trajectory Points"=w43:T27[], "CurrentIndex"=w49:u32)
        n14 = Array Size(array=w44) -> (size(s)=w41:i32)
        n15 = Array Size(array=w43) -> (size(s)=w42:i32)
        n16 = Not Equal To 0?(x=w42) -> (x != 0?=w39:bool)
        n17 = Not Equal To 0?(x=w41) -> (x != 0?=w40:bool)
        n18 = Compound Arithmetic op=AND(w28, w39, w40) -> (w38:bool)
        n19 = case shown="False" w38 {
          tunnel: w53 -> [_ w104]
          tunnel: w52 -> [_ w103]
          tunnel: w51 -> [_ w102]
          tunnel: w50 -> [_ w101]
          tunnel: w49 -> [_ w100]
          tunnel: w48 -> [w57 w96]
          tunnel: w47 -> [w58 w95]
          tunnel: [w58 w85] -> w46
          tunnel: [w57 w83] -> w45
          tunnel: w44 -> [_ w89]
          tunnel: w43 -> [_ w88]
          tunnel: w37 -> [w56 w87]
          tunnel: [w56 w82] -> w36
          tunnel: w29 -> [_ w77]
          tunnel: w30 -> [_ w78]
          tunnel: [w55 w64] -> w35
          tunnel: w34 -> [w55 w62]
          tunnel: w33 -> [_ w61]
          tunnel: w32 -> [_ w60]
          tunnel: w31 -> [_ w59]
          frame False {
            # "No path to follow"
          }
          frame True {
            # "Mark as executing"
            # "Follow Path"
            n20 = Unbundle By Name(w102) -> ("Motors.DriveLeftPrimary.Unit Conversion Factor"=w72:dbl, "Motors.DriveRightPrimary.Unit Conversion Factor"=w71:dbl)  [unwired: 1 out]
            n21 = Bundle By Name(cluster=w77, "CurrentIndex"=u32 1) -> (w74:T25)
            n22 = Bundle By Name(cluster=w78, "CurrentIndex"=u32 1) -> (w73:T25)
            n23 = global write "MotionProfileControlData.vi" "LeftDriveMPControl"(w74) -> ()
            n24 = global write "MotionProfileControlData.vi" "RightDriveMPControl"(w73) -> ()
            n25 = call "ADI_IMU_ADIS16448_Get Angles.vi"("ADI IMU DevRef"=w104) -> ("IMU Angles Out"=w105:T28)  [unwired: 7 in, 3 out]
            n26 = Unbundle By Name(w103) -> ("DriveLeftPrimary"=w80:T21, "DriveRightPrimary"=w79:T21)
            n27 = Unbundle By Name(w105) -> ("Z Angle"=w94:dbl)
            n28 = Equal To 0?(x=w101) -> (x = 0?=w98:bool)
            n29 = Equal To 0?(x=w100) -> (x = 0?=w99:bool)
            n30 = Scale By Power Of 2(n=i16 1, x=w94) -> (x*2^n=w70:dbl)
            n31 = And(x=w98, y=w99) -> (x .and. y?=w97:bool)
            n32 = Tick Count (ms)() -> (millisecond timer value=w81:u32)
            n33 = case shown="False" w97 {
              tunnel: [w182 w184] -> w84
              tunnel: w96 -> [w182 _]
              tunnel: w70 -> [_ w185]
              tunnel: [w181 w185] -> w86
              tunnel: w95 -> [w181 _]
              tunnel: [w180 w183] -> w68
              tunnel: w87 -> [w180 _]
              tunnel: w81 -> [_ w184]
              tunnel: [w179 w183] -> w63
              tunnel: w62 -> [w179 _]
              frame False {
              }
              frame True {
                w183 = FALSE
                # "First Point"
              }
            }
            n34 = for {
              tunnel: w89 -> [w178] mode=indexing
              tunnel: w88 -> [w177] mode=indexing
              tunnel: [w176] -> w90 mode=indexing
              tunnel: [w175] -> w91 mode=indexing
              tunnel: [w174] -> w92 mode=indexing
              tunnel: [w173] -> w93 mode=indexing
              n35 = Unbundle By Name(w178) -> ("velocity"=w176:dbl, "dt"=w175:dbl, "heading"=w174:dbl)
              n36 = Unbundle By Name(w177) -> ("velocity"=w173:dbl)
            }
            n37 = call "EdgeDetector.vi"("DetectorType"=EdgeDetector_Type."RisingEdge", "Input"=w68) -> ("Edge"=w66:bool)
            n38 = case shown="False" w68 {
              selector: w68 -> [_ w164]
              tunnel: w70 -> [w127 _]
              tunnel: w81 -> [w155 _]
              tunnel: w93 -> [w153 _]
              tunnel: w92 -> [w150 _]
              tunnel: w91 -> [w139 _]
              tunnel: w90 -> [w152 _]
              tunnel: [w128 w165] -> w85
              tunnel: w86 -> [w128 w165]
              tunnel: w84 -> [w151 w166]
              tunnel: [w151 w166] -> w83
              tunnel: [w138 w164] -> w82
              tunnel: w80 -> [w136 w163]
              tunnel: w79 -> [w134 w162]
              tunnel: "DriveGyro Kp ((in/sec)/deg)" -> [w148 _]
              tunnel: w72 -> [w146 _]
              tunnel: w71 -> [w145 _]
              tunnel: w66 -> [_ w159]
              tunnel: [w111 w158] -> w64
              tunnel: w63 -> [_ w158]
              tunnel: w61 -> [w109 w161]
              tunnel: w60 -> [w117 _]
              tunnel: w59 -> [w113 _]
              frame False {
                w137 = T29 2 items=["PercentOutput"=0, "Position"=1, "Velocity"=2, "Current"=3, "Follower"=5, "MotionProfile"=6, "MotionMagic"=7, "MotionMagicArc"=8, "MotionProfileArc"=10, "Disabled"=15] ("Control Mode")
                # "End early if motion stopped"
                # "Gyro increases CW,\nPath planner increases CCW"
                # "Convert from ticks/s\nto tics/100ms"
                # "Adjust for heading\nerror"
                # "Use linear interpolation to find\nvelocity and heading at this\ntime sample"
                # "Finished when time after last time"
                # "Not finished yet"
                n39 = Compound Arithmetic op=ADD(invert w151, w155) -> (w142:u32)
                n40 = Array Size(array=w139) -> (size(s)=w141:i32)
                n41 = call "DeltaAngle_Degrees.vi"("EndAngle (deg)"=w127, "StartAngle (deg)"=w128) -> ("DeltaAngle (deg)"=w124:dbl)
                n42 = Divide(x=w142, y=u32 1000) -> (x/y=w106:dbl)
                n43 = Decrement(x=w141) -> (x-1=w140:i32)
                n44 = call "Lookup_Table.vi"("Y_Array"=w152, "x_in"=w106, "X_Array"=w139) -> ("y_out"=w144:dbl)  [unwired: 6 in]
                n45 = call "Lookup_Table.vi"("Y_Array"=w150, "x_in"=w106, "X_Array"=w139) -> ("y_out"=w125:dbl)  [unwired: 6 in]
                n46 = call "Lookup_Table.vi"("Y_Array"=w153, "x_in"=w106, "X_Array"=w139) -> ("y_out"=w143:dbl)  [unwired: 6 in]
                n47 = Negate(x=w124) -> (-x=w122:dbl)
                n48 = Index Array(array=w139, index=w140) -> (element=w107:dbl)
                n49 = Index Array(array=w150) -> (element=w126:dbl)  [unwired: 1 in]
                n50 = Greater Or Equal?(x=w106, y=w107) -> (x >= y?=w138:bool)
                n51 = call "DeltaAngle_Degrees.vi"("EndAngle (deg)"=w125, "StartAngle (deg)"=w126) -> ("DeltaAngle (deg)"=w123:dbl)
                n52 = call "DeltaAngle_Degrees.vi"("EndAngle (deg)"=w123, "StartAngle (deg)"=w122) -> ("DeltaAngle (deg)"=w149:dbl)
                n53 = Divide(x=w106, y=w107) -> (x/y=w114:dbl)
                n54 = Multiply(x=w149, y=w148) -> (x*y=w147:dbl)
                n55 = Greater Or Equal?(x=w114, y=w113) -> (x >= y?=w112:bool)
                n56 = Subtract(x=w144, y=w147) -> (x-y=w121:dbl)
                n57 = Subtract(x=w143, y=w147) -> (x-y=w118:dbl)
                n58 = Absolute Value(x=w121) -> (abs(x)=w120:dbl)
                n59 = Absolute Value(x=w118) -> (abs(x)=w119:dbl)
                n60 = Less?(x=w120, y=w117) -> (x < y?=w115:bool)
                n61 = Less?(x=w119, y=w117) -> (x < y?=w116:bool)
                n62 = Multiply(x=w146, y=w121) -> (x*y=w135:dbl)
                n63 = Multiply(x=w145, y=w118) -> (x*y=w133:dbl)
                n64 = Compound Arithmetic op=AND(w112, w115, w116) -> (w111:bool)
                n65 = call "EdgeDetector.vi"("DetectorType"=EdgeDetector_Type."RisingEdge", "Input"=w111) -> ("Edge"=w108:bool)
                n66 = case shown="True" w108 {
                  tunnel: w109 -> [_ w156]
                  frame False {
                  }
                  frame True {
                    n67 = Send Notification(notification=TRUE, notifier=w156) -> ()  [unwired: 1 in, 2 out]
                  }
                }
                n68 = Divide(x=w135, y=10.0) -> (x/y=w132:dbl)
                n69 = Divide(x=w133, y=10.0) -> (x/y=w130:dbl)
                n70 = call <vilib>:"CTRE_Phoenix_MotorControl_Set.vi"("Output"=w132, "Control Mode"=w137, "PhoenixMotorControlDevRef"=w136) -> ()  [unwired: 7 in, 2 out]
                n71 = call <vilib>:"CTRE_Phoenix_MotorControl_Set.vi"("Output"=w130, "Control Mode"=w137, "PhoenixMotorControlDevRef"=w134) -> ()  [unwired: 7 in, 2 out]
              }
              frame True {
                # "Only set 0 velocity once"
                # "Completed path already, so skip most of the calculations"
                n72 = Compound Arithmetic op=AND(invert w158, w159) -> (w160:bool)
                n73 = case shown="True" w160 {
                  tunnel: w163 -> [_ w171]
                  tunnel: w162 -> [_ w170]
                  tunnel: w161 -> [_ w167]
                  frame False {
                  }
                  frame True {
                    w169 = 0.0 ("Output")
                    w172 = T29 2 items=["PercentOutput"=0, "Position"=1, "Velocity"=2, "Current"=3, "Follower"=5, "MotionProfile"=6, "MotionMagic"=7, "MotionMagicArc"=8, "MotionProfileArc"=10, "Disabled"=15] ("Control Mode")
                    n74 = Send Notification(notification=TRUE, notifier=w167) -> ()  [unwired: 1 in, 2 out]
                    n75 = call <vilib>:"CTRE_Phoenix_MotorControl_Set.vi"("Output"=w169, "Control Mode"=w172, "PhoenixMotorControlDevRef"=w171) -> ()  [unwired: 7 in, 2 out]
                    n76 = call <vilib>:"CTRE_Phoenix_MotorControl_Set.vi"("Output"=w169, "Control Mode"=w172, "PhoenixMotorControlDevRef"=w170) -> ()  [unwired: 7 in, 2 out]
                  }
                }
              }
            }
          }
        }
      }
    }
    n77 = call <vilib>:"Release Semaphore.vi"("semaphore"=w25) -> ()  [unwired: 5 in, 2 out]
  }
